vi "test.vi"() -> ()   [LabVIEW 2016]
uses:
  Source/JSON Value/Variant Support/JSFL Variant Support.lvlib
panel:
  out "data":cluster{"String":string}
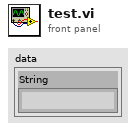
[diagram p1: front panel]
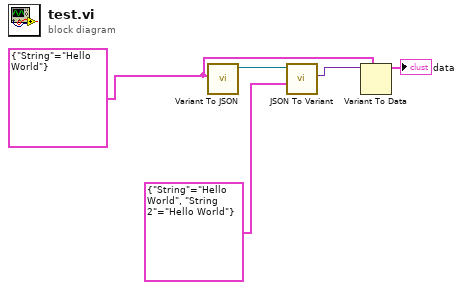
[diagram p0: block diagram]
diagram:
  w2 = cluster{"String":string} {"String"="Hello World"}
  n1 = call "Variant To JSON.vi"("Variant"=w2) -> ("JSON Value out"=w5:refnum<class "JSON Value.lvclass">)  [unwired: 9 in, 1 out]
  n2 = call "JSON To Variant.vi"("datatype and defaults"=cluster{"String":string, "String 2":string} {"String"="Hello World", "String 2"="Hello World"}, "JSON Value in"=w5) -> ("Variant"=w4:variant)  [unwired: 8 in, 1 out]
  n3 = Variant To Data(type=w2, Variant=w4) -> (data=→"data":cluster{"String":string})  [unwired: 1 in, 1 out]
